vi "OpenG Array filter - Regexp Array Template.vi"() -> ()   [LabVIEW 2012]
panel:
  out "filtered item indices":i32[](array[numeric])
  out "filtered array":string[](array[string])
  in  "items to filter":string[](array[string])
  in  "Array Input":string[](array[string])
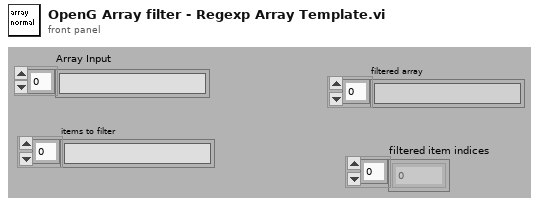
[diagram p1: front panel]
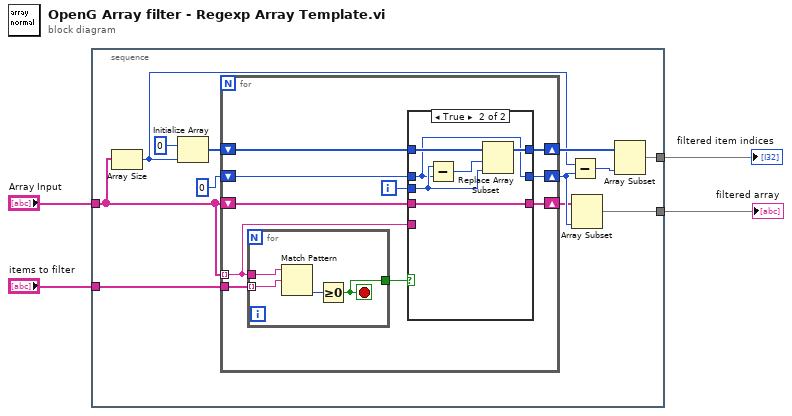
[diagram p0: block diagram]
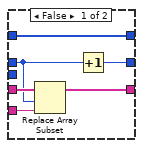
[diagram p2: hidden frame]
diagram:
  n1 = stacked-sequence {
    tunnel: "items to filter" -> [w7]
    tunnel: [w5] -> w3
    tunnel: "Array Input" -> [w8]
    tunnel: [w6] -> w1
    frame #0 {
      n2 = Array Size(array=w8) -> (size(s)=w13:i32)
      n3 = Initialize Array(0 ("Numeric"), w13) -> (w12:i32[])
      n4 = for {
        tunnel: w8 -> [w23] mode=indexing
        shift-right: [w24] -> w10
        shift-left: w8 -> [w26]
        shift-right: [w21] -> w15
        shift-left: 0 -> [w22]
        shift-right: [w19] -> w14
        shift-left: w12 -> [w20]
        tunnel: w7 -> [w18]
        i -> [w17]
        n5 = for {
          tunnel: [w29] -> w25
          tunnel: w23 -> [w28]
          tunnel: w18 -> [w27] mode=indexing
          stop <- w29 stop-if-true
          n6 = Match Pattern(string=w28, regular expression=w27) -> (offset past match=w30:i32)  [unwired: 4 out]
          n7 = Greater Or Equal To 0?(x=w30) -> (x >= 0?=w29:bool)
        }
        n8 = case shown="True" w25 {
          tunnel: w26 -> [w36 w42]
          tunnel: [w35 w42] -> w24
          tunnel: w23 -> [w34 _]
          tunnel: w22 -> [w32 w38]
          tunnel: [w33 w38] -> w21
          tunnel: w20 -> [w31 w41]
          tunnel: [w31 w40] -> w19
          tunnel: w17 -> [_ w39]
          frame False {
            n9 = Replace Array Subset(array=w36, new element=w34, index=w32) -> (w35:string[])
            n10 = Increment(x=w32) -> (x+1=w33:i32)
          }
          frame True {
            n11 = Subtract(x=w39, y=w38) -> (x-y=w37:i32)
            n12 = Replace Array Subset(array=w41, new element=w39, index=w37) -> (w40:i32[])
          }
        }
      }
      n13 = Subtract(x=w13, y=w15) -> (x-y=w16:i32)
      n14 = Array Subset(array=w10, length=w15) -> (w6:string[])  [unwired: 1 in]
      n15 = Array Subset(array=w14, length=w16) -> (w5:i32[])  [unwired: 1 in]
    }
  }
  "filtered array" <- w1
  "filtered item indices" <- w3
